vi "Launcher.vi"() -> ()   [LabVIEW 2020]
doc: "このVIを実行します。"
uses:
  support/Message Queue/Message Queue.lvlib
  Loop/UI/UI.lvlib
  support/User Event - Stop/User Event - Stop.lvlib
panel:
  out "error out":errorcluster
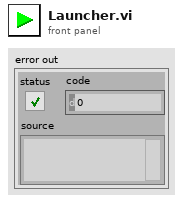
[diagram p1: front panel]
types:
  T1 = enum32{"Invalid", "Standard", "Closed", "Hidden", "Minimized", "Maximized"}
  T2 = typedef "Message Queue.lvlib/All Message Queues.ctl" = cluster{"UI":refnum<queue>}
  T3 = typedef "User Event - Stop.lvlib/User Events.ctl" = cluster{"Stop":refnum<user-event>}
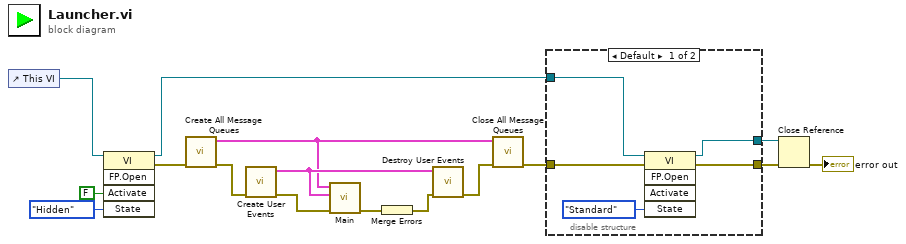
[diagram p0: block diagram]
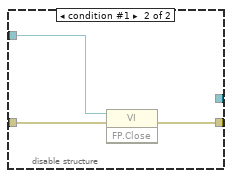
[diagram p2: hidden frame]
diagram:
  n1 = control-ref of="This VI"() -> (w12:refnum<vi>)
  n2 = invoke class="VI" method="FP.Open"(reference=w12, "Activate"=FALSE ("Activate?"), "State"=T1."Hidden") -> (reference out=w8:refnum<vi>, error out=w9:errorcluster)  [unwired: 2 in, 3 out]
  n3 = call "Create All Message Queues.vi"("error in (no error)"=w9) -> ("error out"=w15:errorcluster, "Message Queues out"=w1:T2)  [unwired: 9 in]
  n4 = call "Create User Events.vi"("error in (no error)"=w15) -> ("error out"=w3:errorcluster, "User Events"=w2:T3)  [unwired: 9 in]
  n5 = call "Main.vi"("error in"=w3, "User Events"=w2, "Message Queues in"=w1) -> ("error out"=w16:errorcluster)  [unwired: 8 in]
  n6 = Merge Errors(w16) -> (w14:errorcluster)
  n7 = call "Destroy User Events.vi"("error in (no error)"=w14, "User Events"=w2) -> ("error out"=w13:errorcluster)  [unwired: 9 in]
  n8 = call "Close All Message Queues.vi"("error in (no error)"=w13, "Message Queues"=w1) -> ("error out"=w7:errorcluster)  [unwired: 9 in]
  n9 = disable-structure shown="Default" {
    disable-tunnel: w8 -> [w21 w24]
    disable-tunnel: w7 -> [w20 w23]
    disable-tunnel: [w18 w22] -> w6
    disable-tunnel: [w17 _] -> w5
    frame condition #0 (active) {
      n10 = invoke class="VI" method="FP.Open"(reference=w21, error in=w20, "State"=T1."Standard") -> (reference out=w17:refnum<vi>, error out=w18:errorcluster)  [unwired: 2 in, 3 out]
    }
    frame condition #1 {
      n11 = invoke class="VI" method="FP.Close"(reference=w24, error in=w23) -> (error out=w22:errorcluster)  [unwired: 1 in, 2 out]
    }
  }
  n12 = Close Reference(reference=w5, error in (no error)=w6) -> (error out=→"error out":errorcluster)
